vi "VIH HelpGen - Get VI Conpane Image.vi"(8 "error in":errorcluster, 9 "Get Icon if no Conpane Image (F)":bool, 10 "Enable Check (T)":bool=TRUE, 11 "VI Reference":refnum<vi>) -> (0 "error out":errorcluster, 2 "Conpane Image":T1, 3 "dup VI Reference":refnum<vi>)   [LabVIEW 2014]
doc: "::: VI Helpeks :::\nCopyright (c) 2000-2026 Konstantin Shifershteyn. All rights reserved."
uses:
  <vilib>/picture/picture.llb/imagedata.ctl
panel:
  # "VI Helpeks\nCopyright (c) 2012-2026 Konstantin Shifershteyn"
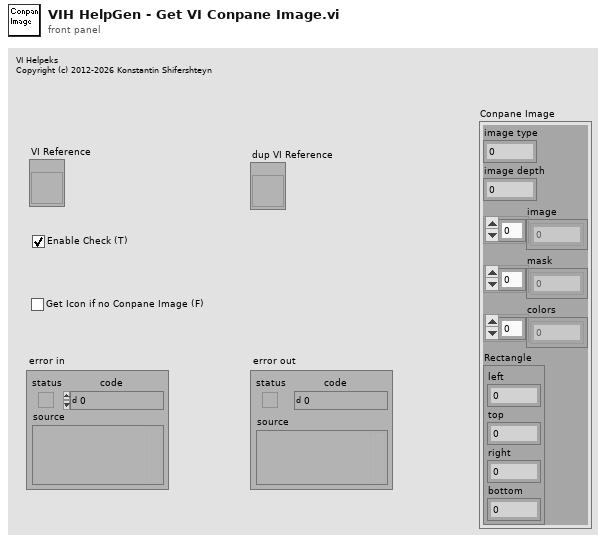
[diagram p1: front panel]
types:
  T1 = typedef "imagedata.ctl" = cluster{"image type":i32, "image depth":i32, "image":u8[], "mask":u8[], "colors":u32[], "Rectangle":cluster{"left":i16, "top":i16, "right":i16, "bottom":i16}}
  T2 = enum16{"Invalid Wire Rule", "Required", "Recommended", "Optional", "Dynamic Dispatch"}
  T3 = enum16{"Invalid Wire Rule", "Required", "Recommended", "Optional", "Dynamic Dispatch"}[]
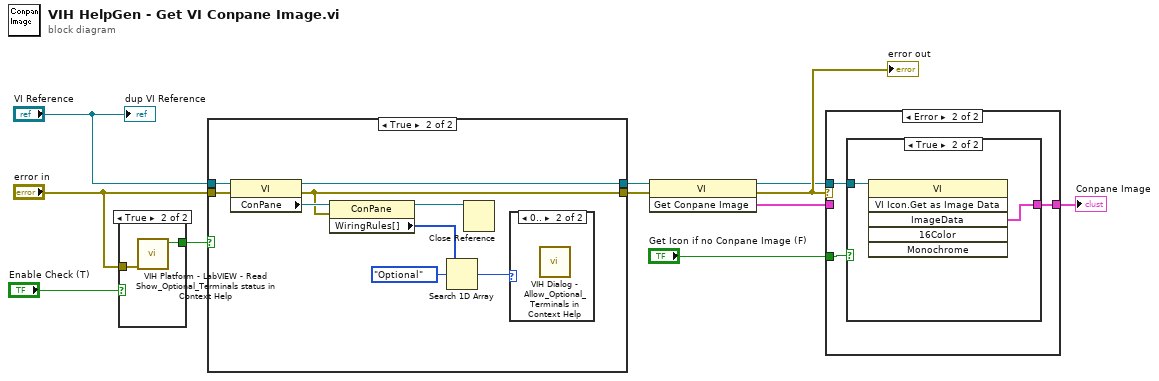
[diagram p0: block diagram]
diagram:
  n1 = case shown="True" "Enable Check (T)" {
    tunnel: [_ w13] -> w11
    tunnel: "error in" -> [_ w12]
    frame False {
    }
    frame True {
      n2 = call "VIH Platform - LabVIEW - Read Show_Optional_Terminals status in Context Help.vi"("error in"=w12) -> ("simpleDiagramHelp (Hide Optional Terminals)"=w13:bool)  [unwired: 9 in, 1 out]
    }
  }
  n3 = case shown="True" w11 {
    tunnel: "error in" -> [w14 w19]
    tunnel: "VI Reference" -> [w15 w20]
    tunnel: [w15 w17] -> w8
    tunnel: [w14 w16] -> w7
    frame False {
    }
    frame True {
      n4 = property class="VI"(reference=w20, error in=w19) -> (reference out=w17:refnum<vi>, error out=w16:errorcluster, "ConPane"=w24:refnum<vi>)
      n5 = property class="ConPane"(reference=w24, error in=w16) -> (reference out=w21:refnum<vi>, "WiringRules[]"=w23:T3)  [unwired: 1 out]
      n6 = Search 1D Array(1D array=w23, element=T2."Optional") -> (index of element=w18:i32)  [unwired: 1 in]
      n7 = Close Reference(reference=w21) -> ()  [unwired: 1 in, 1 out]
      n8 = case shown="0.." w18 {
        frame ..-1 {
        }
        frame 0.. {
          n9 = call "VIH Dialog - Allow_Optional_Terminals in Context Help.vi"() -> ()  [unwired: 11 in, 1 out]
        }
      }
    }
  }
  n10 = invoke class="VI" method="Get Conpane Image"(reference=w8, error in=w7) -> (reference out=w2:refnum<vi>, error out=w5:errorcluster, "Get Conpane Image"=w4:T1)  [unwired: 1 in]
  "error out" <- w5
  n11 = case shown="Error" w5 {
    tunnel: w4 -> [w25 _]
    tunnel: [w25 w27] -> w3
    tunnel: w2 -> [_ w28]
    tunnel: "Get Icon if no Conpane Image (F)" -> [_ w26]
    frame No Error {
    }
    frame Error {
      n12 = case shown="True" w26 {
        tunnel: w28 -> [_ w30]
        tunnel: [_ w29] -> w27
        frame False {
        }
        frame True {
          n13 = invoke class="VI" method="VI Icon.Get as Image Data"(reference=w30) -> ("ImageData"=w29:T1)  [unwired: 5 in, 5 out]
        }
      }
    }
  }
  "Conpane Image" <- w3
  "dup VI Reference" <- "VI Reference"
